vi "TF Customer.vi"   [LabVIEW 2020]
uses:
  builds/Source Distributions/Triarc Framework/Triarc Framework/Process/Process.lvclass
  Documents/GitHub/Triarc-Examples/Coffee Shop/Processes/People/Customers/Customer/Customer.lvclass
  builds/Source Distributions/Triarc Framework/Triarc Framework/View/View.lvclass
  Documents/GitHub/Triarc-Examples/Coffee Shop/Support/Beverages/Beverage/Beverage.lvclass
  C:/Git/astemes-triarc-framework/builds/Source Distributions/Triarc Framework/Triarc Framework/Base/Base.lvclass
  C:/Git/astemes-triarc-framework/builds/Source Distributions/Triarc Framework/Triarc Framework/Process/Process.lvclass
  C:/Git/astemes-triarc-framework/builds/Source Distributions/Triarc Framework/Triarc Framework/Error Handler Interface/Error Handler Interface.lvclass
  C:/Git/astemes-triarc-framework/builds/Source Distributions/Triarc Framework/Triarc Framework/Logging/Logging.lvclass
  C:/Git/astemes-triarc-framework/builds/Source Distributions/Triarc Framework/Triarc Framework/View/View.lvclass
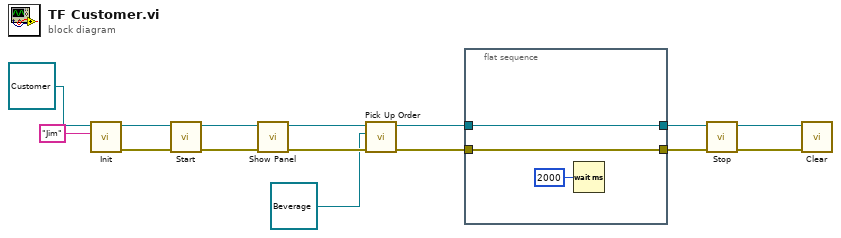
[diagram p0: block diagram]
diagram:
  n1 = call-dynamic "Init.vi"("Name"="Jim", "View In"=refnum<class "Customer.lvclass"> refnum ("Customer.lvclass")) -> ("error out"=w14:errorcluster, "View Out"=w15:refnum<class "Customer.lvclass">)  [unwired: 8 in]
  n2 = call "Start.vi"("error in (no error)"=w14, "Process In"=w15) -> ("error out"=w13:errorcluster, "Process Out"=w8:refnum<class "Process.lvclass">)  [unwired: 7 in, 1 out]
  n3 = call "Show Panel.vi"("error in (no error)"=w13, "View In"=w8) -> ("error out"=w9:errorcluster, "View Out"=w7:refnum<class "View.lvclass">)  [unwired: 8 in]
  n4 = call "Pick Up Order.vi"("error in (no error)"=w9, "Beverage.lvclass"=refnum<class "Beverage.lvclass"> refnum, "Customer in"=w7) -> ("error out"=w5:errorcluster, "Customer out"=w2:refnum<class "Customer.lvclass">)  [unwired: 7 in]
  n5 = flat-sequence {
    tunnel: [w17] -> w4
    tunnel: w5 -> [w17]
    tunnel: [w16] -> w3
    tunnel: w2 -> [w16]
    frame #0 {
      n6 = Wait (ms)(milliseconds to wait=u32 2000) -> ()  [unwired: 1 out]
    }
  }
  n7 = call "Stop.vi"("error in (no error)"=w4, "Process In"=w3) -> ("error out"=w11:errorcluster, "Process Out"=w12:refnum<class "Process.lvclass">)  [unwired: 7 in, 1 out]
  n8 = call-dynamic "Clear.vi"("error in (no error)"=w11, "Process In"=w12) -> ()  [unwired: 9 in, 1 out]
